vi "CANsub_REST_Setup.vi"(6 "bit timing":T1={"brp"=2, "seg1"=63, "seg2"=16, "sjw"=16, "data brp"=2, "data seg1"=15, "data seg2"=4, "data sjw"=4}, 7 "phase":T2, 8 "error in (no error)":errorcluster, 9 "cert path":path=path "/home/lvuser/cansub_root_cert.crt", 10 "channel":u8=2, 11 "host":string) -> (0 "error out":errorcluster, 3 "api version":string)   [LabVIEW 2021, in "CANsub_Common.lvlib"]
doc: "CANsub channel setup over REST. before_ws: checks API version 05.00 and that the channel is stopped, deletes old filters and transmit sequences, sets the bit timing (with TX acknowledgements and error frames). after_ws: adds the two accept-all filters; without them the device sends no frames. TLS without server verification (bench limitation). Error 5000: HTTP status; 5001: API version; 5002: channel busy."
uses:
  CANsub_Common.lvlib
  <vilib>/httpClient/LabVIEWHTTPClient.lvlib
  Typedefs/HTTP_Method.ctl
  Typedefs/REST_Phase.ctl
  Typedefs/Bit_Timing.ctl
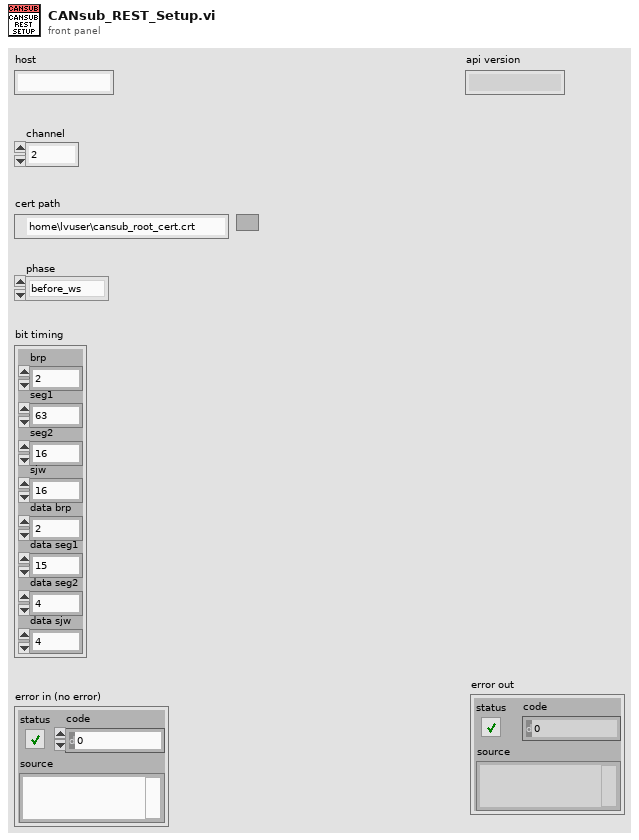
[diagram p1: front panel]
types:
  T1 = typedef "CANsub_Common.lvlib/Bit_Timing.ctl" = cluster{"brp":u16, "seg1":u16, "seg2":u16, "sjw":u16, "data brp":u16, "data seg1":u16, "data seg2":u16, "data sjw":u16}
  T2 = typedef "CANsub_Common.lvlib/REST_Phase.ctl" = enum16{"before_ws", "after_ws"}
  T3 = typedef "LabVIEWHTTPClient.lvlib/ClientHandle.ctl" = refnum<k1>
  T4 = typedef "CANsub_Common.lvlib/HTTP_Method.ctl" = enum16{"GET", "PUT", "POST", "DELETE"}
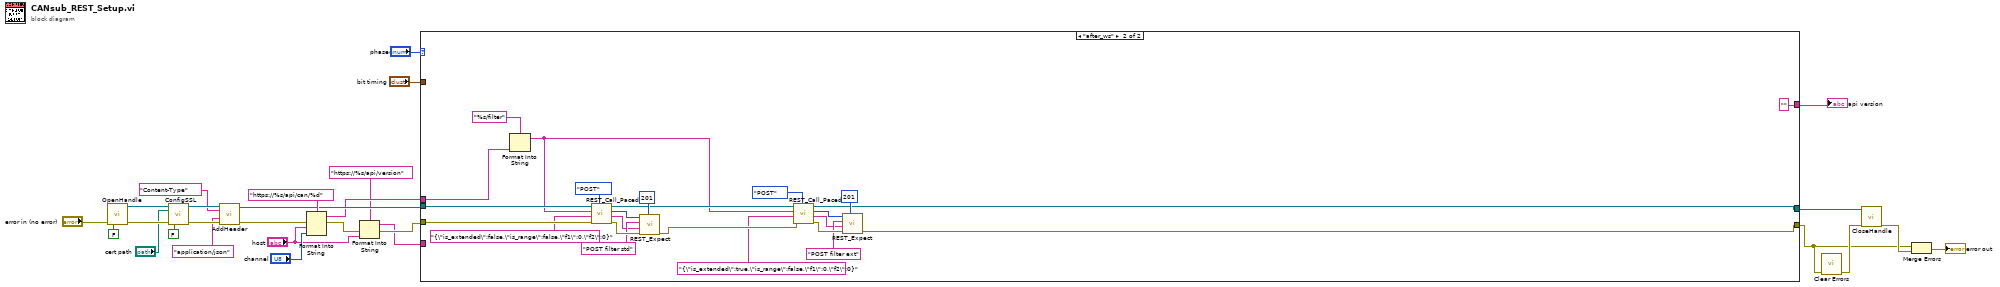
[diagram p0: block diagram]
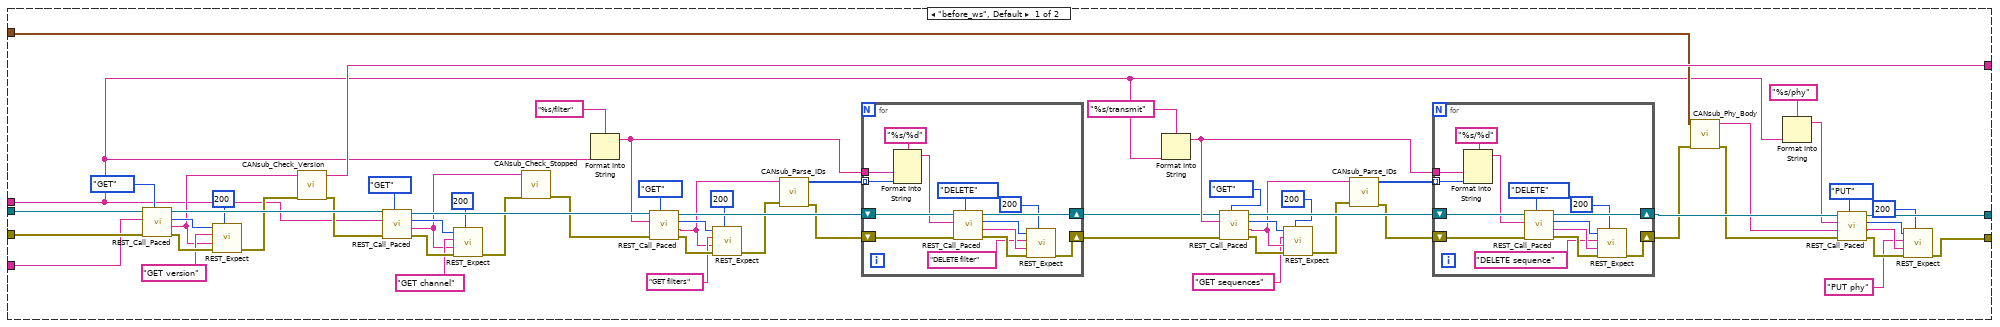
[diagram p2: hidden frame]
diagram:
  n1 = call <vilib>:"OpenHandle.vi"("error in (no error)"="error in (no error)", "verify server(true)"=FALSE) -> ("client handle out"=w18:T3, "error out"=w21:errorcluster)  [unwired: 12 in]
  n2 = call <vilib>:"ConfigSSL.vi"("client handle"=w18, "CA certificate file"="cert path", "error in (no error)"=w21, "verify server (true)"=FALSE) -> ("client handle out"=w17:T3, "error out"=w23:errorcluster)  [unwired: 10 in]
  n3 = call <vilib>:"AddHeader.vi"("client handle"=w17, "header"="Content-Type", "value"="application/json", "error in (no error)"=w23) -> ("client handle out"=w16:T3, "error out"=w19:errorcluster)  [unwired: 10 in]
  n4 = Format Into String(format string="https://%s/api/can/%d", error in=w19, "host", "channel") -> (resulting string=w14:string, error out=w3:errorcluster)  [unwired: 1 in]
  n5 = Format Into String(format string="https://%s/api/version", error in=w3, "host") -> (resulting string=w1:string, error out=w2:errorcluster)  [unwired: 1 in]
  n6 = case shown="\"after_ws\"" "phase" {
    tunnel: w2 -> [w86 w131]
    tunnel: w16 -> [w85 w132]
    tunnel: [w32 w122] -> w8
    tunnel: w14 -> [w30 w129]
    tunnel: [w81 w123] -> w10
    tunnel: [w72 "" ("api version")] -> w7
    tunnel: "bit timing" -> [w41 _]
    tunnel: w1 -> [w31 _]
    frame "before_ws", Default {
      n7 = call "REST_Call_Paced.vi"("method"=HTTP_Method."GET", "error in (no error)"=w86, "url"=w31, "client handle"=w85) -> ("error out"=w92:errorcluster, "response"=w75:string, "status"=w80:i32, "client handle out"=w84:T3)  [unwired: 4 in]
      n8 = call "REST_Expect.vi"("expected"=200, "error in (no error)"=w92, "response"=w75, "what"="GET version", "status"=w80) -> ("error out"=w74:errorcluster)  [unwired: 5 in, 1 out]
      n9 = call "CANsub_Check_Version.vi"("error in (no error)"=w74, "response"=w75) -> ("error out"=w73:errorcluster, "api version"=w72:string)  [unwired: 8 in]
      n10 = call "REST_Call_Paced.vi"("method"=HTTP_Method."GET", "error in (no error)"=w73, "url"=w30, "client handle"=w84) -> ("error out"=w91:errorcluster, "response"=w64:string, "status"=w76:i32, "client handle out"=w83:T3)  [unwired: 4 in]
      n11 = call "REST_Expect.vi"("expected"=200, "error in (no error)"=w91, "response"=w64, "what"="GET channel" ("response"), "status"=w76) -> ("error out"=w70:errorcluster)  [unwired: 5 in, 1 out]
      n12 = call "CANsub_Check_Stopped.vi"("error in (no error)"=w70, "response"=w64) -> ("error out"=w69:errorcluster)  [unwired: 7 in, 2 out]
      n13 = Format Into String(format string="%s/filter", w30) -> (resulting string=w57:string)  [unwired: 2 in, 1 out]
      n14 = call "REST_Call_Paced.vi"("method"=HTTP_Method."GET", "error in (no error)"=w69, "url"=w57, "client handle"=w83) -> ("error out"=w90:errorcluster, "response"=w61:string, "status"=w62:i32, "client handle out"=w82:T3)  [unwired: 4 in]
      n15 = call "REST_Expect.vi"("expected"=200, "error in (no error)"=w90, "response"=w61, "what"="GET filters", "status"=w62) -> ("error out"=w60:errorcluster)  [unwired: 5 in, 1 out]
      n16 = call "CANsub_Parse_IDs.vi"("error in (no error)"=w60, "response"=w61) -> ("error out"=w59:errorcluster, "ids"=w58:i32[])  [unwired: 8 in]
      n17 = for {
        shift-right: [w118] -> w43
        shift-left: w59 -> [w120]
        shift-right: [w115] -> w44
        shift-left: w82 -> [w116]
        tunnel: w58 -> [w112] mode=indexing
        tunnel: w57 -> [w113]
        n18 = Format Into String(format string="%s/%d", w113, w112) -> (resulting string=w111:string)  [unwired: 2 in, 1 out]
        n19 = call "REST_Call_Paced.vi"("method"=HTTP_Method."DELETE", "error in (no error)"=w120, "url"=w111, "client handle"=w116) -> ("error out"=w119:errorcluster, "response"=w109:string, "status"=w110:i32, "client handle out"=w115:T3)  [unwired: 4 in]
        n20 = call "REST_Expect.vi"("expected"=200, "error in (no error)"=w119, "response"=w109, "what"="DELETE filter", "status"=w110) -> ("error out"=w118:errorcluster)  [unwired: 5 in, 1 out]
      }
      n21 = Format Into String(format string="%s/transmit", w30) -> (resulting string=w49:string)  [unwired: 2 in, 1 out]
      n22 = call "REST_Call_Paced.vi"("method"=HTTP_Method."GET", "error in (no error)"=w43, "url"=w49, "client handle"=w44) -> ("error out"=w56:errorcluster, "response"=w53:string, "status"=w54:i32, "client handle out"=w55:T3)  [unwired: 4 in]
      n23 = call "REST_Expect.vi"("expected"=200, "error in (no error)"=w56, "response"=w53, "what"="GET sequences", "status"=w54) -> ("error out"=w52:errorcluster)  [unwired: 5 in, 1 out]
      n24 = call "CANsub_Parse_IDs.vi"("error in (no error)"=w52, "response"=w53) -> ("error out"=w51:errorcluster, "ids"=w50:i32[])  [unwired: 8 in]
      n25 = for {
        shift-right: [w104] -> w40
        shift-left: w51 -> [w106]
        shift-right: [w101] -> w42
        shift-left: w55 -> [w102]
        tunnel: w50 -> [w98] mode=indexing
        tunnel: w49 -> [w99]
        n26 = Format Into String(format string="%s/%d", w99, w98) -> (resulting string=w97:string)  [unwired: 2 in, 1 out]
        n27 = call "REST_Call_Paced.vi"("method"=HTTP_Method."DELETE", "error in (no error)"=w106, "url"=w97, "client handle"=w102) -> ("error out"=w105:errorcluster, "response"=w95:string, "status"=w96:i32, "client handle out"=w101:T3)  [unwired: 4 in]
        n28 = call "REST_Expect.vi"("expected"=200, "error in (no error)"=w105, "response"=w95, "what"="DELETE sequence", "status"=w96) -> ("error out"=w104:errorcluster)  [unwired: 5 in, 1 out]
      }
      n29 = call "CANsub_Phy_Body.vi"("error in (no error)"=w40, "Bit_Timing"=w41) -> ("error out"=w39:errorcluster, "body"=w37:string)  [unwired: 8 in]
      n30 = Format Into String(format string="%s/phy", w30) -> (resulting string=w36:string)  [unwired: 2 in, 1 out]
      n31 = call "REST_Call_Paced.vi"("method"=HTTP_Method."PUT", "error in (no error)"=w39, "body"=w37, "url"=w36, "client handle"=w42) -> ("error out"=w89:errorcluster, "response"=w34:string, "status"=w35:i32, "client handle out"=w81:T3)  [unwired: 3 in]
      n32 = call "REST_Expect.vi"("expected"=200, "error in (no error)"=w89, "response"=w34, "what"="PUT phy", "status"=w35) -> ("error out"=w32:errorcluster)  [unwired: 5 in, 1 out]
    }
    frame "after_ws" {
      n33 = Format Into String(format string="%s/filter", w129) -> (resulting string=w125:string)  [unwired: 2 in, 1 out]
      n34 = call "REST_Call_Paced.vi"("method"=HTTP_Method."POST", "error in (no error)"=w131, "body"="{\"is_extended\":false,\"is_range\":false,\"f1\":0,\"f2\":0}", "url"=w125, "client handle"=w132) -> ("error out"=w144:errorcluster, "response"=w139:string, "status"=w142:i32, "client handle out"=w127:T3)  [unwired: 3 in]
      n35 = call "REST_Expect.vi"("expected"=201, "error in (no error)"=w144, "response"=w139, "what"="POST filter std", "status"=w142) -> ("error out"=w126:errorcluster)  [unwired: 5 in, 1 out]
      n36 = call "REST_Call_Paced.vi"("method"=HTTP_Method."POST", "error in (no error)"=w126, "body"="{\"is_extended\":true,\"is_range\":false,\"f1\":0,\"f2\":0}", "url"=w125, "client handle"=w127) -> ("error out"=w138:errorcluster, "response"=w133:string, "status"=w136:i32, "client handle out"=w123:T3)  [unwired: 3 in]
      n37 = call "REST_Expect.vi"("expected"=201, "error in (no error)"=w138, "response"=w133, "what"="POST filter ext", "status"=w136) -> ("error out"=w122:errorcluster)  [unwired: 5 in, 1 out]
    }
  }
  "api version" <- w7
  n38 = call <vilib>:"Clear Errors.vi"("error in (no error)"=w8) -> ("error out"=w25:errorcluster)  [unwired: 5 in, 1 out]
  n39 = call <vilib>:"CloseHandle.vi"("client handle"=w10, "error in (no error)"=w25) -> ("error out"=w15:errorcluster)  [unwired: 13 in]
  n40 = Merge Errors(w8, w15) -> (→"error out":errorcluster)
